vi "ArchiveDirectory Value Change.vi"(4 "Linux Archive Directory":string caption="Archive Directory", 6 "Windows Archive Directory":path, 7 "Control Refs":T1, 9 "Linux Paths?":bool, 10 "Event References":T2, 11 "References":T9) -> (0 "error out":errorcluster)   [LabVIEW 2015, in "TDMS datalogger editor node.lvclass"]
uses:
  TDMS datalogger editor node.lvclass
  <vilib>/NI/DCAF/Tag Editor Core/Table API/Table Manager/object ref.ctl
  <vilib>/NI/DCAF/Tag Editor Core/Configuration Editor/Classes/Engine Parent/Engine Parent Editor Node.lvclass
  <vilib>/NI/DCAF/Tag Editor Core/Configuration Editor/Classes/Module editor node/module editor node.lvclass
  <vilib>/NI/DCAF/Tag Editor Core/Table API/Table Manager/references.ctl
  <vilib>/NI/Configuration Framework/Node/StopEvent.ctl
  <vilib>/NI/Configuration Framework/Node/RefreshUIEvent.ctl
  <vilib>/NI/Configuration Framework/Node/CacheState.ctl
  <vilib>/NI/Configuration Framework/Node/NodeChangeEvent.ctl
  <vilib>/NI/Configuration Framework/Node/NodeRef.ctl
  <vilib>/NI/Configuration Framework/Node/NISE_CEF_Node.lvclass
  <vilib>/NI/DCAF/Tag Editor Core/Table API/Available Tag Menu/channel action event.ctl
  <vilib>/NI/DCAF/Tag Editor Core/Table API/Available Tag Menu/dialog output action.ctl
  <vilib>/NI/Tag Bus Module Framework/channel/TBM channel.lvclass
  <vilib>/NI/Tag Bus/tag/tag descriptor.lvclass
  <vilib>/NI/DCAF/Tag Editor Core/Table API/Table Manager/Call Back Ref Type Def.ctl
  <vilib>/NI/AMC/Message Queue.ctl
  <vilib>/NI/AMC/Message.ctl
  <vilib>/NI/Tools/Keyed Array/KeyedArray.ctl
  <vilib>/NI/Configuration Framework/Node/UserEventRef.ctl
  <vilib>/NI/Configuration Framework/Controls/EventCluster.ctl
  Control Refs.ctl
  TDMS datalogger editor node.lvclass/TDMS datalogger editor node.ctl
  module/configuration/TDMS datalogger configuration.lvclass/TDMS datalogger configuration.ctl
  module/configuration/Write backup directory.vi
  module/configuration/TDMS datalogger configuration.lvclass
  <vilib>/NI/DCAF/Tag Editor Core/Table API/Table Manager/Table Manager.lvclass
  <vilib>/NI/DCAF/Tag Editor Core/Table API/Table Manager.lvlib
  <vilib>/NI/Tools/Keyed Array/Tools_KeyedArray.lvlib
  <vilib>/NI/AMC/AMC.lvlib
  <vilib>/NI/Configuration Framework/NISE_CEF_TreeControl.lvlib
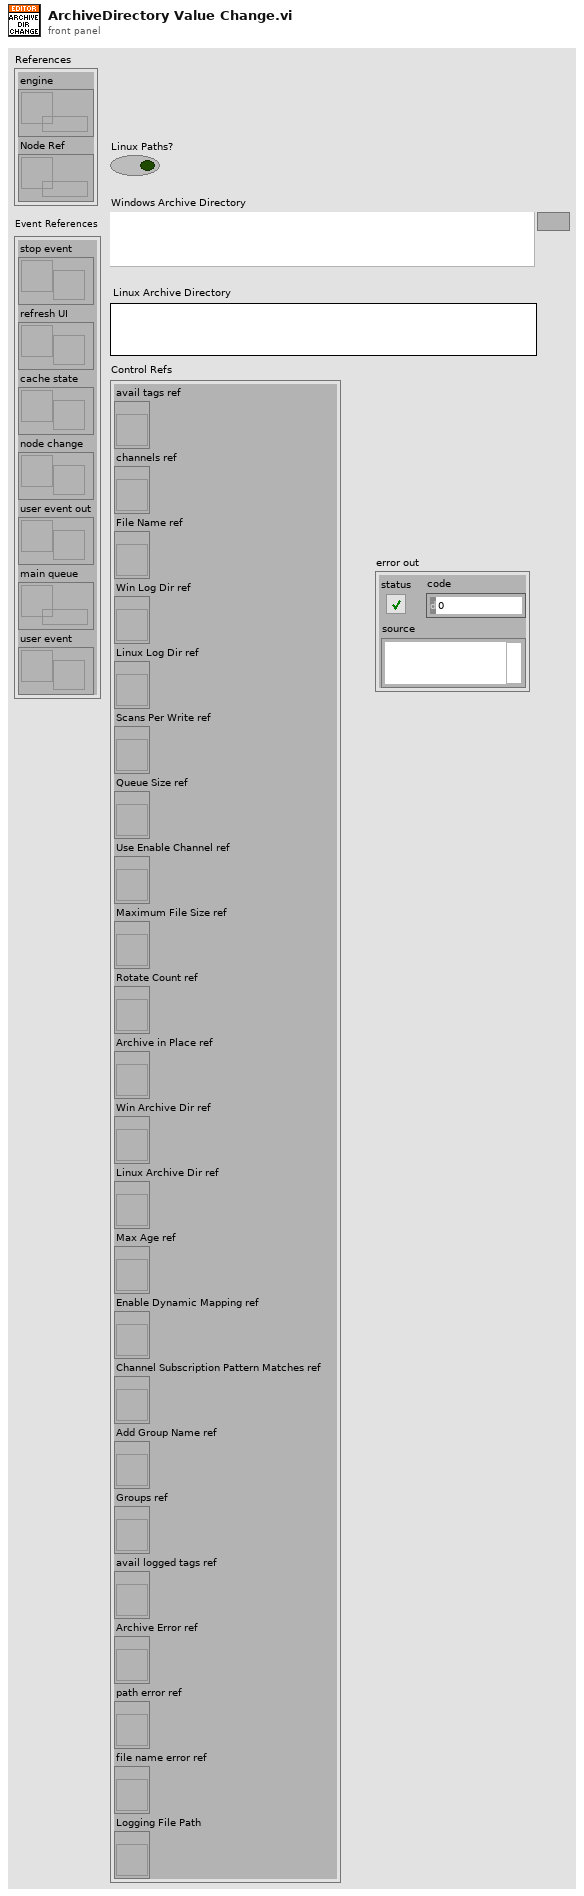
[diagram p1: front panel]
types:
  T1 = typedef "Control Refs.ctl" = cluster{"avail tags ref":refnum<vi>, "channels ref":refnum<vi>, "File Name ref":refnum<vi>, "Win Log Dir ref":refnum<vi>, "Linux Log Dir ref":refnum<vi>, "Scans Per Write ref":refnum<vi>, "Queue Size ref":refnum<vi>, "Use Enable Channel ref":refnum<vi>, "Maximum File Size ref":refnum<vi>, "Rotate Count ref":refnum<vi>, "Archive in Place ref":refnum<vi>, "Win Archive Dir ref":refnum<vi>, "Linux Archive Dir ref":refnum<vi>, "Max Age ref":refnum<vi>, "Enable Dynamic Mapping ref":refnum<vi>, "Channel Subscription Pattern Matches ref":refnum<vi>, "Add Group Name ref":refnum<vi>, "Groups ref":refnum<vi>, "avail logged tags ref":refnum<vi>, "Archive Error ref":refnum<vi>, "path error ref":refnum<vi>, "file name error ref":refnum<vi>, "Logging File Path":refnum<vi>}
  T2 = typedef "Table Manager.lvlib/Table Manager.lvclass/references.ctl" = cluster{"stop event":T3, "refresh UI":T4, "cache state":T5, "node change":T6, "user event out":refnum<user-event>, "main queue":T7, "user event":T8}
  T3 = typedef "NISE_CEF_Node.lvclass/StopEvent.ctl" = refnum<user-event>
  T4 = typedef "NISE_CEF_Node.lvclass/RefreshUIEvent.ctl" = refnum<user-event>
  T5 = typedef "NISE_CEF_Node.lvclass/CacheState.ctl" = refnum<user-event>
  T6 = typedef "NISE_CEF_Node.lvclass/NodeChangeEvent.ctl" = refnum<user-event>
  T7 = typedef "AMC.lvlib/Message Queue.ctl" = refnum<queue>
  T8 = typedef "NISE_CEF_Node.lvclass/UserEventRef.ctl" = refnum<user-event>
  T9 = typedef "Table Manager.lvlib/Table Manager.lvclass/object ref.ctl" = cluster{"engine":refnum<data-value>, "Node Ref":refnum<data-value>}
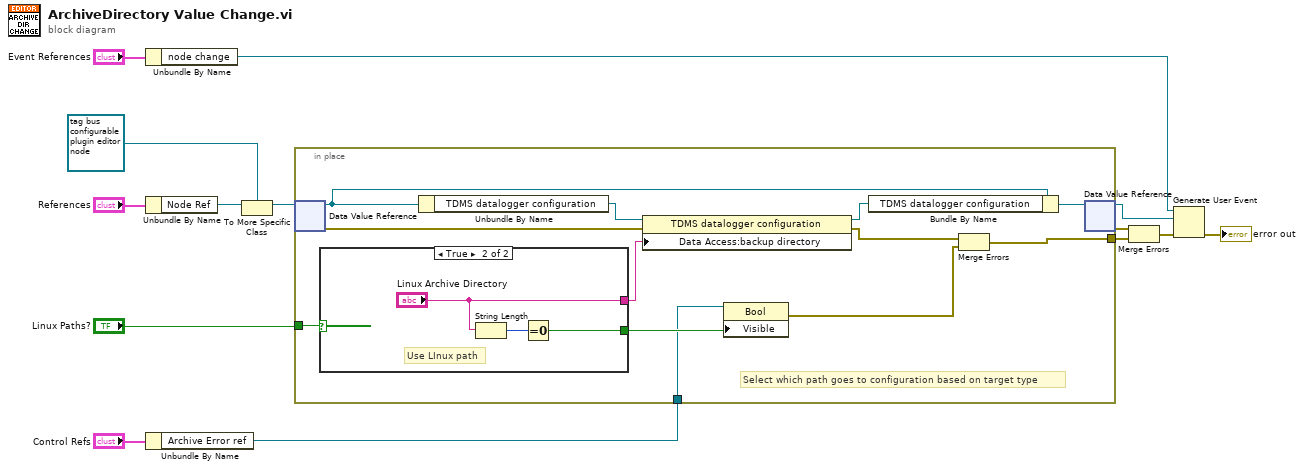
[diagram p0: block diagram]
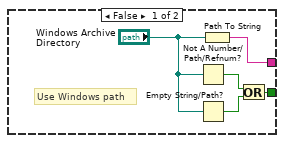
[diagram p2: hidden frame]
diagram:
  n1 = Unbundle By Name("Event References") -> ("node change"=w4:T6)
  n2 = Unbundle By Name("References") -> ("Node Ref"=w13:refnum<data-value>)
  n3 = Unbundle By Name("Control Refs") -> ("Archive Error ref"=w1:refnum<vi>)
  n4 = To More Specific Class(target class=refnum<data-value> refnum ("data value reference"), reference=w13) -> (specific class reference=w10:refnum<data-value>)  [unwired: 1 in, 1 out]
  n5 = in-place {
    in-place-border: [w16] -> w8
    in-place-border: "Linux Paths?" -> [w18]
    in-place-border: w1 -> [w17]
    # "Select which path goes to configuration based on target type"
    n6 = in-place-dvr #1(w10) -> (w25:refnum<class "TDMS datalogger editor node.lvclass">, w20:errorcluster)
    n7 = case shown="True" w18 {
      tunnel: [w28 w32] -> w24
      tunnel: [w27 "Linux Archive Directory"] -> w19
      frame False {
        # "Use Windows path"
        n8 = Not A Number/Path/Refnum?(number/path/refnum="Windows Archive Directory") -> (NaN/Path/Refnum?=w30:bool)
        n9 = Empty String/Path?(string/path="Windows Archive Directory") -> (empty?=w31:bool)
        n10 = Path To String(path="Windows Archive Directory") -> (string=w27:string)
        n11 = Or(x=w30, y=w31) -> (x .or. y?=w28:bool)
      }
      frame True {
        # "Use LInux path"
        n12 = String Length(string="Linux Archive Directory") -> (length=w33:i32)
        n13 = Equal To 0?(x=w33) -> (x = 0?=w32:bool)
      }
    }
    n14 = Unbundle By Name(w25) -> ("TDMS datalogger configuration"=w21:refnum<class "TDMS datalogger configuration.lvclass">)
    n15 = property class="TDMS datalogger configuration"(reference=w21, error in=w20, "Data Access:backup directory"=w19) -> (reference out=w22:refnum<class "TDMS datalogger configuration.lvclass">, error out=w23:errorcluster)
    n16 = property on="Property Node" class="Bool"(reference=w17, "Visible"=w24) -> (error out=w15:errorcluster)  [unwired: 1 in, 1 out]
    n17 = Bundle By Name(cluster=w25, "TDMS datalogger configuration"=w22) -> (w26:refnum<class "TDMS datalogger editor node.lvclass">)
    n18 = Merge Errors(w23, w15) -> (w16:errorcluster)
    n19 = in-place-dvr #1(w26) -> (w3:refnum<data-value>, w7:errorcluster)
  }
  n20 = Merge Errors(w7, w8) -> (w6:errorcluster)
  n21 = Generate User Event(user event=w4, event data cluster=w3, error in=w6) -> (error out=→"error out":errorcluster)  [unwired: 1 in, 1 out]
